vi "{TMPL} MAIN - App.vi"() -> ()   [LabVIEW 2022 SP3, in "TLB` Template.lvlib" / "{TMPL} TLB`.lvclass"]
uses:
  {TMPL} TLB`.lvclass
  Application Components/Trigger API/System Trigger.ctl
  State Machine/State.ctl
  Core Components/Error Handler/TLB` Error Handler.lvclass
  Application Components/Configuration/{TMPL} Station Configuration.lvclass
  {TMPL} TLB`.lvclass/{TMPL} TLB`.ctl
  <vilib>/Utility/error.llb/Error Cluster From Error Code.vi
  <vilib>/ErrorRing/Error Ring.xnode
  Application Components/Trigger API/{TMPL} Trigger API.lvlib
  TLB` Template.lvlib
  Core Components/Actions/Actions.lvlib
  Core Components/Dependencies/TLB`_Dependencies.lvlib
panel:
  out "Banner Text":bool
  in  "Preferences Button":bool=TRUE
  out "Waveform Graph - Light":dbl[](graph)
  in  "Main Tab":T1(tab)
  out "error out":errorcluster
  in  "Connect Instrument":bool
  in  "Disconnect Instrument":bool
  in  "Initiate Analysis":bool
  in  "Stop Analysis":bool
  in  "Load Configuration":bool
  in  "Save Configuration":bool
  in  "Exit":bool
  in  "Active Tab Selector":i32(listbox)
  out "State":string="<Shutdown> "
  out "Status":string
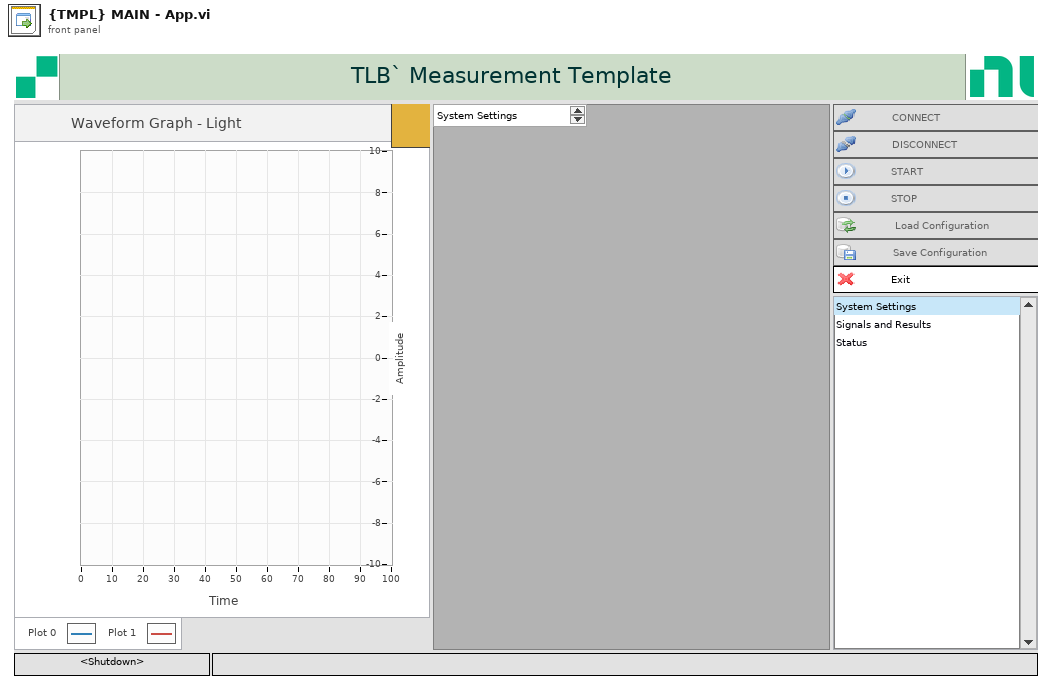
[diagram p1: front panel]
types:
  T1 = enum32{"System Settings", "Signals and Results", "Status"}
  T2 = typedef "TLB` Template.lvlib/{TMPL} TLB`.lvclass/State.ctl" = enum16{"<Startup>", "Idle", "Connected", "Monitoring", "<Shutdown>", "<Error>"}
  T3 = enum16{"Close Display", "Clear References", "Close Error Handler"}
  T4 = enum16{"Clear SR", "Set Display", "Set Shifter", "Initialize Events", "Init Q"}
  T5 = typedef "TLB` Template.lvlib/{TMPL} Trigger API.lvlib/System Trigger.ctl" = enum16{"<None>", "Connect", "Start Acquisition", "Stop Acquisition", "Disconnect", "Load Configuration", "Save Configuration", "<Return to Safe State Actions>", "<Cache User Parameters>", "<Close Application>", "<Error>"}
  T6 = refnum<class "{TMPL} Station Configuration.lvclass">
  T7 = typedef "TLB` Template.lvlib/_UI CORE Event References.ctl" = cluster{"Exit Event":refnum<user-event>, "State Indicator":refnum<user-event>, "Status Indicator":refnum<user-event>}
  T8 = typedef "TLB` Template.lvlib/_UI APP Event References.ctl" = cluster{"Exit Event":refnum<user-event>}
  T9 = enum32{"Invalid", "Standard", "Closed", "Hidden", "Minimized", "Maximized"}
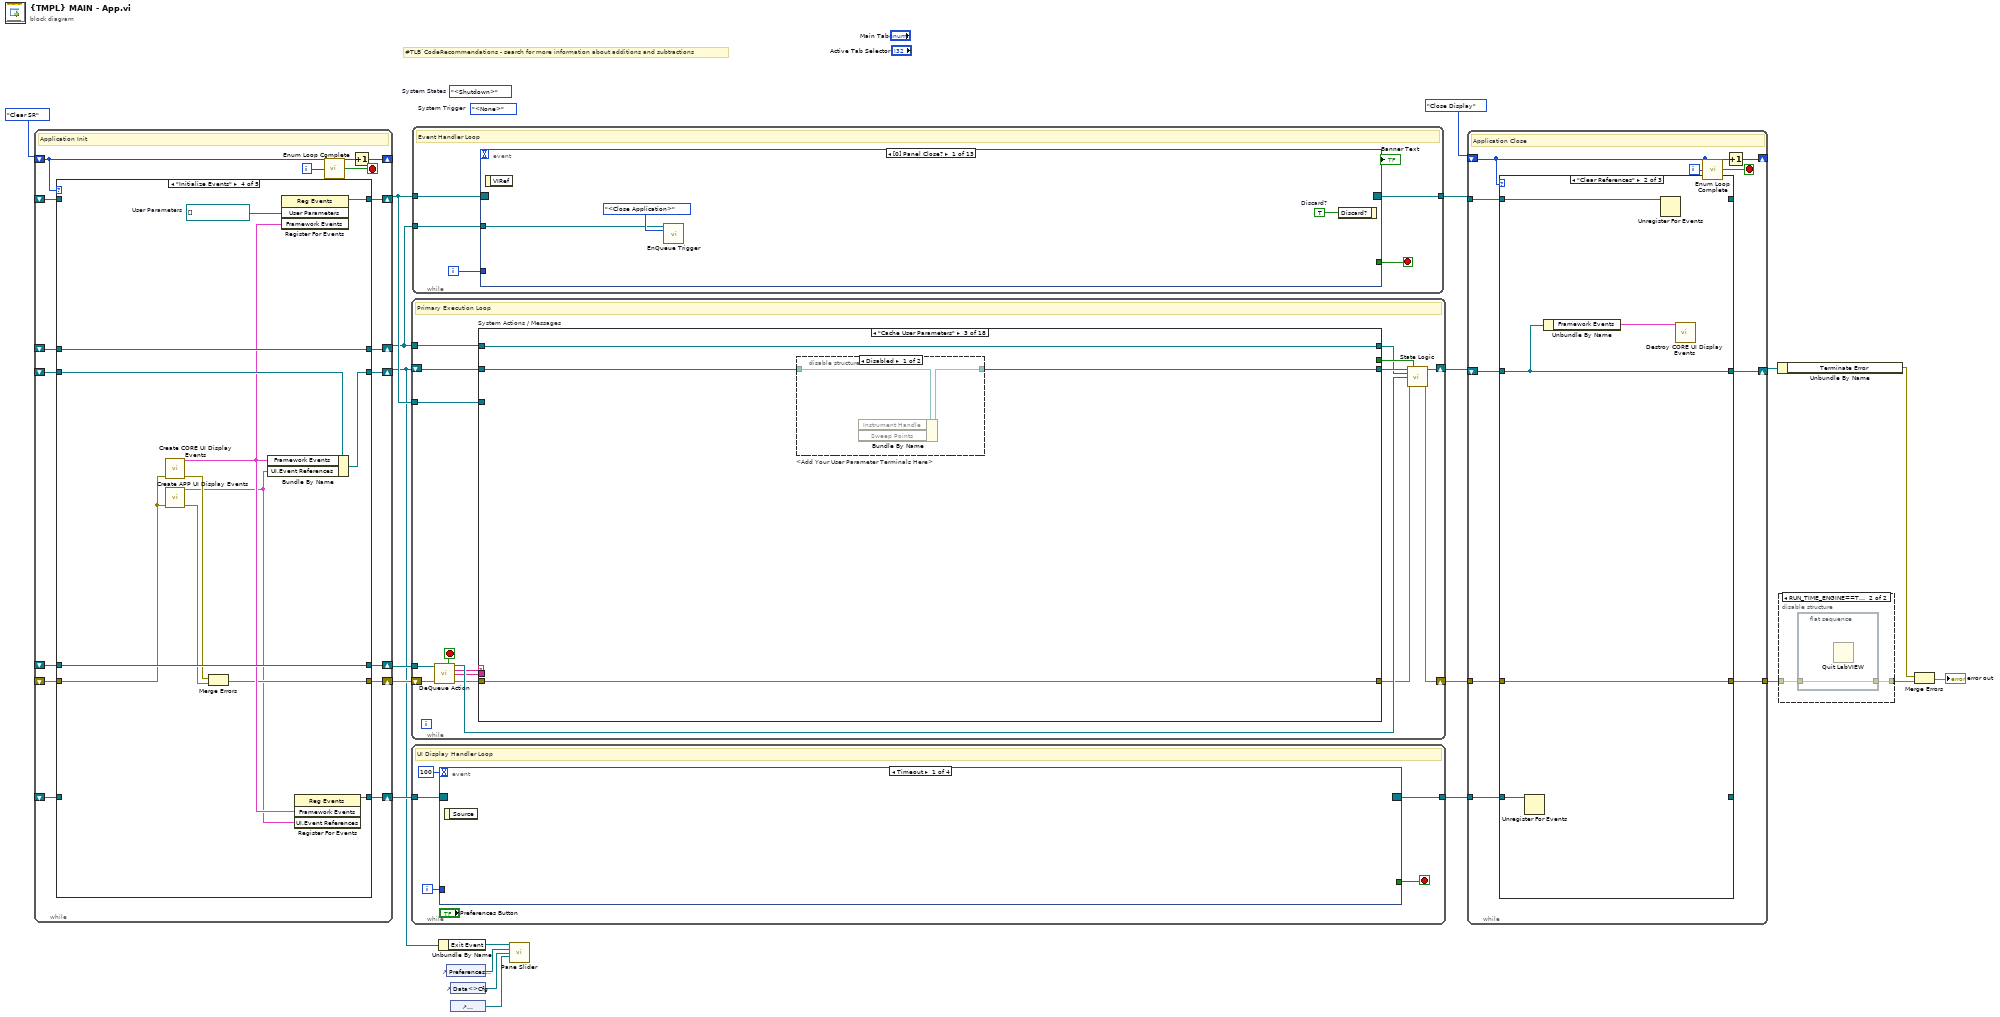
[diagram p0: block diagram]
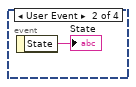
[diagram p2: hidden frame]
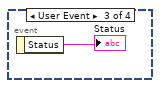
[diagram p3: hidden frame]
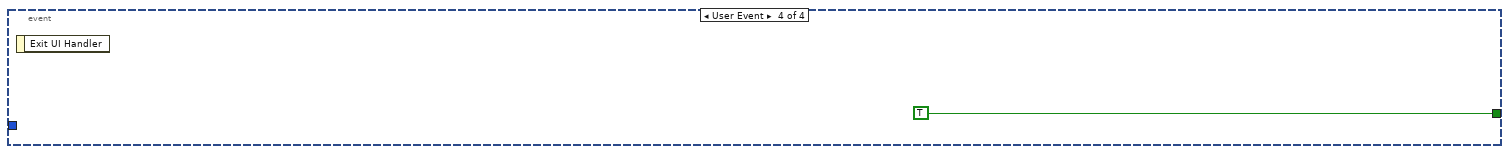
[diagram p4: hidden frame]
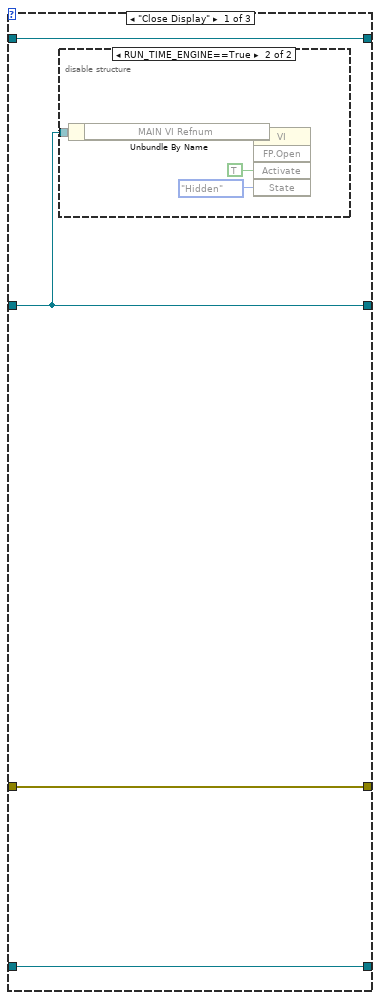
[diagram p6: hidden frame]
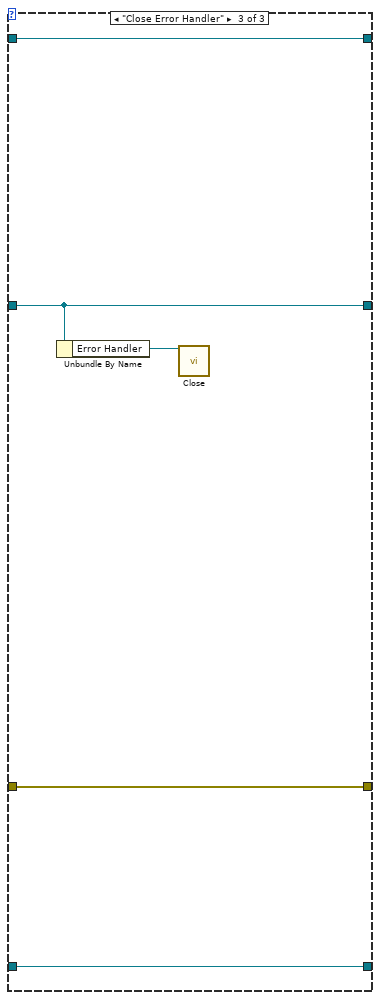
[diagram p8: hidden frame]
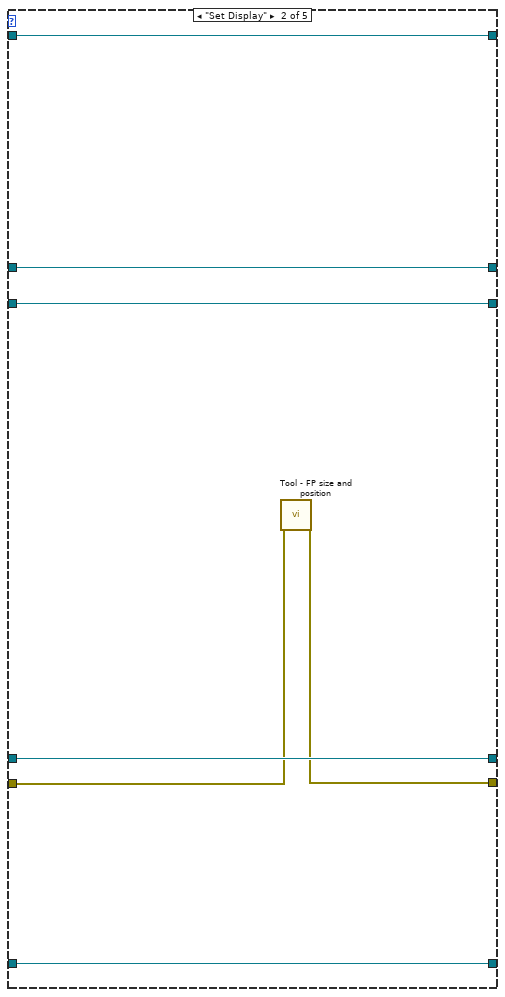
[diagram p10: hidden frame]
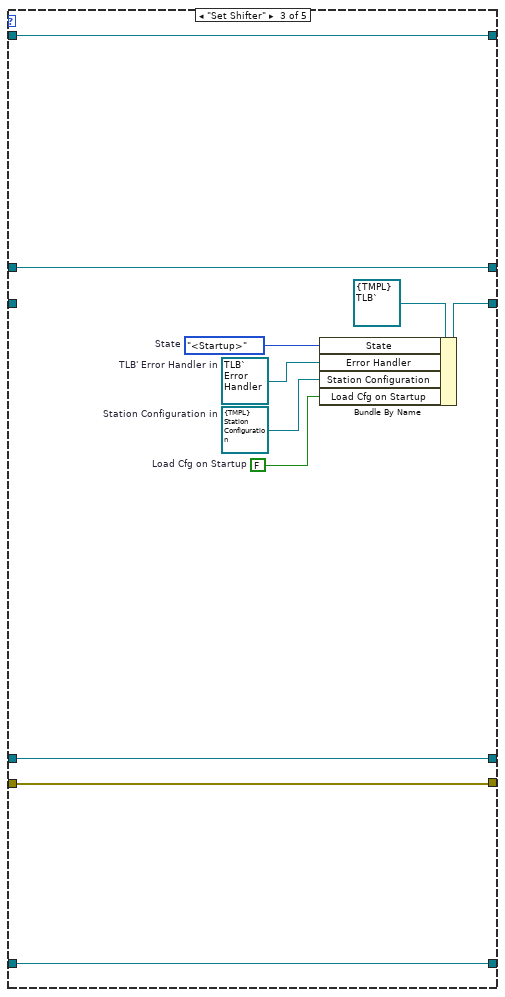
[diagram p11: hidden frame]
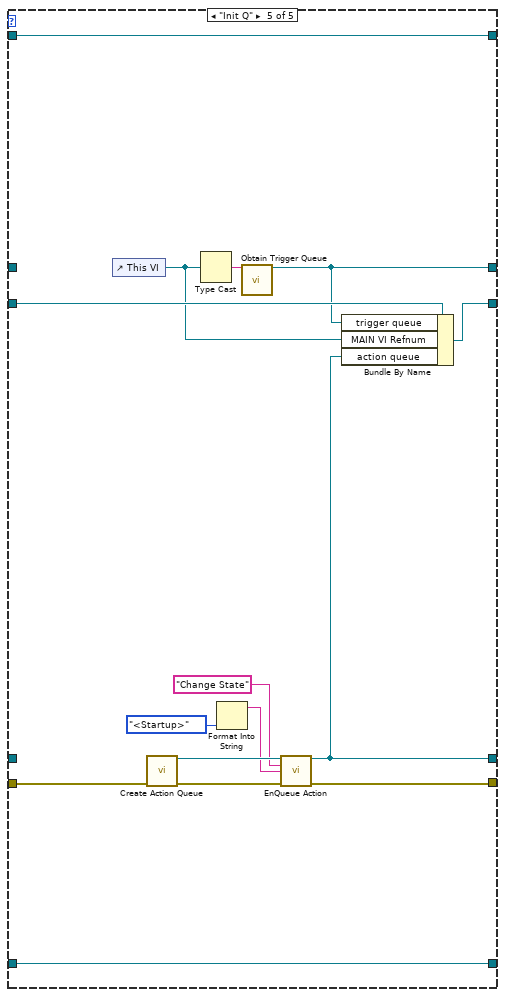
[diagram p12: hidden frame]
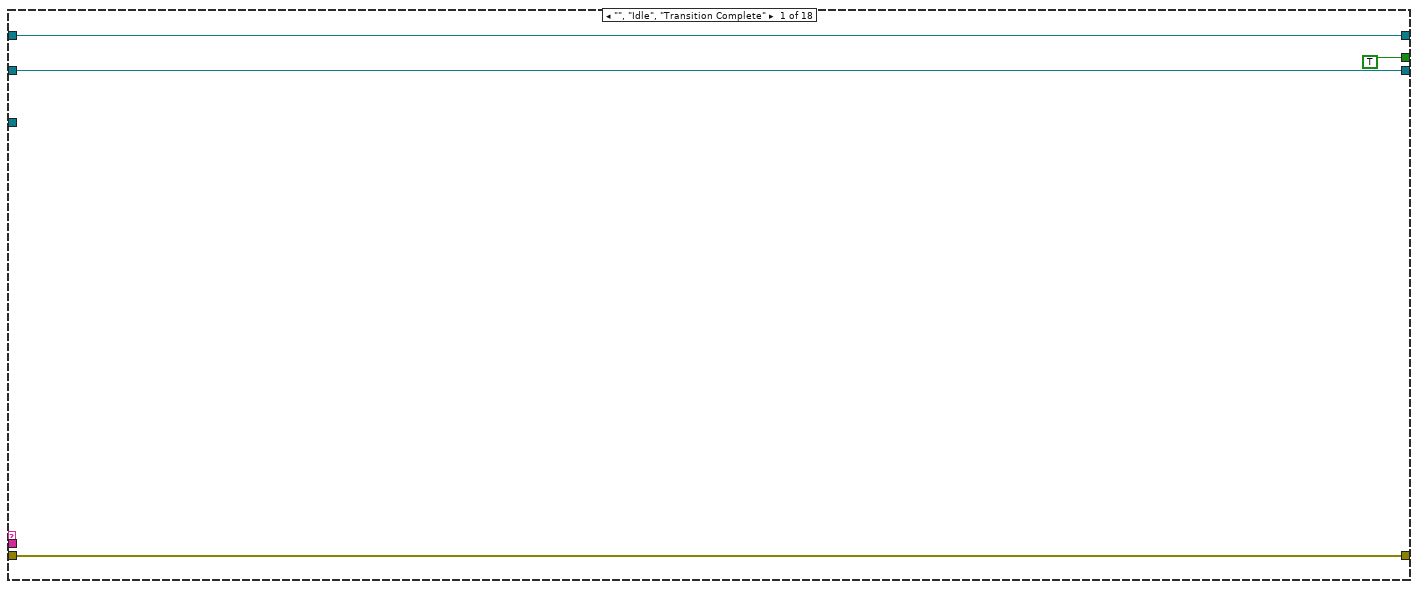
[diagram p13: hidden frame]
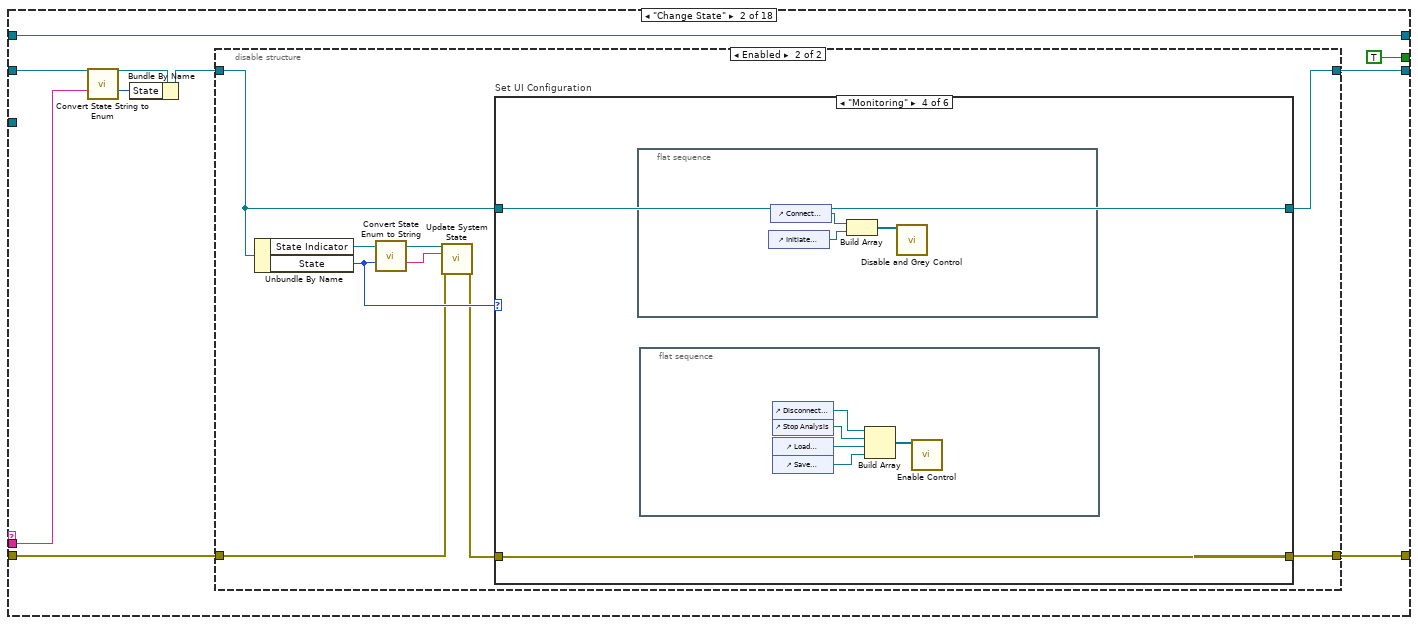
[diagram p14: hidden frame]
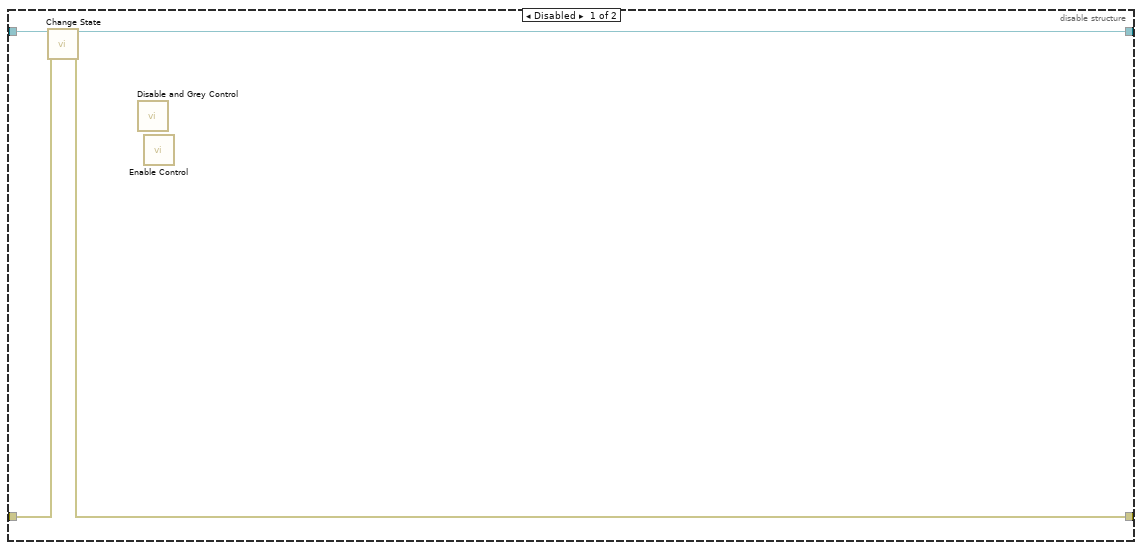
[diagram p15: hidden frame]
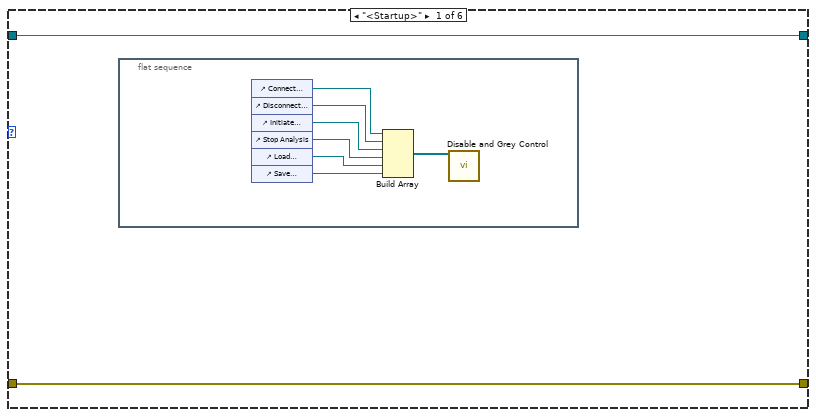
[diagram p16: hidden frame]
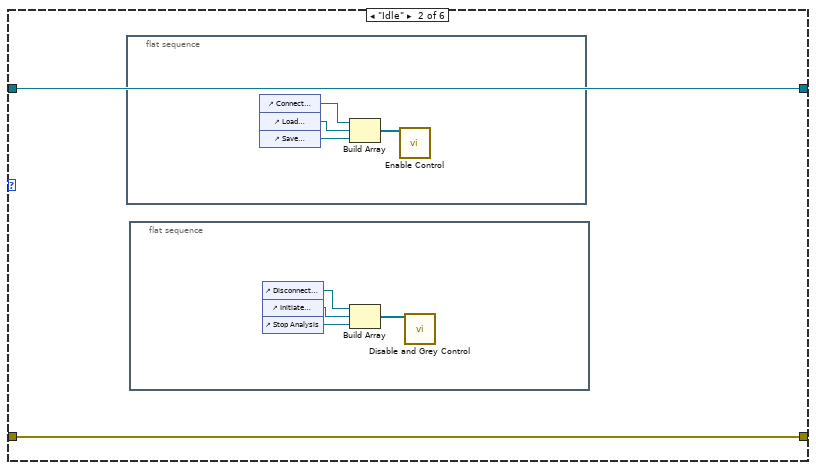
[diagram p17: hidden frame]
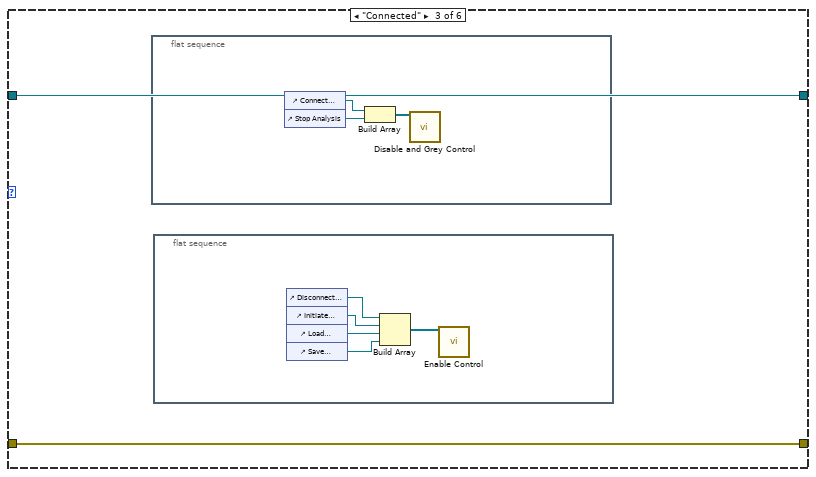
[diagram p18: hidden frame]
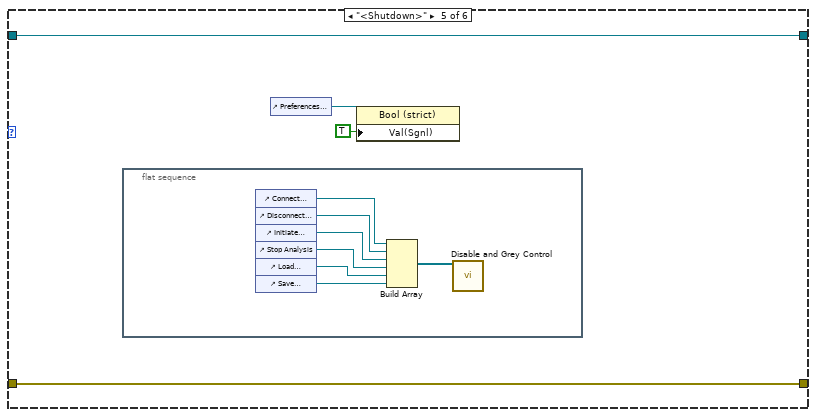
[diagram p19: hidden frame]
diagram:
  (unwired) State."<Shutdown>"  # System States
  (unwired) System_Trigger."<None>"  # System Trigger
  # "#TLB`CodeRecommendations - search for more information about additions and subtractions"
  n1 = while {
    shift-right: [w33] -> _
    shift-left: T4."Clear SR" -> [w22]
    shift-right: [w37] -> w21
    shift-left: _ -> [w32]
    shift-right: [w34] -> w16
    shift-left: _ -> [w31]
    shift-right: [w36] -> w15
    shift-left: _ -> [w30]
    shift-right: [w35] -> w5
    shift-left: _ -> [w29]
    shift-right: [w28] -> w11
    shift-left: _ -> [w27]
    shift-right: [w26] -> w14
    shift-left: _ -> [w25]
    i -> [w23]
    stop <- w24 stop-if-true
    # "Application Init"
    n2 = case shown="\"Initialize Events\"" w22 {
      tunnel: [_ w42 w55 w68 w69] -> w37
      tunnel: [_ w40 w54 w58 w75] -> w34
      tunnel: [_ w44 w50 w66 w81] -> w35
      tunnel: [_ w43 w53 w65 w83] -> w36
      tunnel: w32 -> [_ w42 w55 w68 _]
      tunnel: w31 -> [_ w41 w54 w57 w77]
      tunnel: w30 -> [_ w43 w53 _ w83]
      tunnel: w29 -> [_ w44 _ w67 w82]
      tunnel: [_ w39 w52 w64 w70] -> w28
      tunnel: w27 -> [_ w39 w52 w64 _]
      tunnel: [_ w38 w48 w62 w78] -> w26
      tunnel: w25 -> [_ w38 w48 _ w78]
      frame "Clear SR" {
      }
      frame "Set Display" {
        n3 = call "Tool - FP size and position.vi"("error in (no error)"=w41) -> ("error out"=w40:errorcluster)  [unwired: 17 in, 1 out]
      }
      frame "Set Shifter" {
        w45 = FALSE  # Load Cfg on Startup
        w46 = T6 refnum  # Station Configuration in
        w47 = refnum<class "TLB` Error Handler.lvclass"> refnum  # TLB' Error Handler in
        w51 = State."<Startup>"  # State
        n4 = Bundle By Name(cluster=refnum<class "{TMPL} TLB`.lvclass"> refnum ("TLB` Template.lvlib:TLB' Template.lvclass"), "State"=w51, "Error Handler"=w47, "Station Configuration"=w46, "Load Cfg on Startup"=w45) -> (w50:refnum<class "{TMPL} TLB`.lvclass">)
      }
      frame "Initialize Events" {
        w63 = refnum<vi>[] []  # User Parameters
        n5 = call "Create CORE UI Display Events.vi"("error in"=w57) -> ("Framework Events"=w61:T7, "error out"=w60:errorcluster)  [unwired: 13 in]
        n6 = call "Create APP UI Display Events.vi"("error in"=w57) -> ("UI.Event References"=w56:T8, "error out"=w59:errorcluster)  [unwired: 13 in]
        n7 = Merge Errors(w60, w59) -> (w58:errorcluster)
        n8 = Bundle By Name(cluster=w67, "Framework Events"=w61, "UI.Event References"=w56) -> (w66:refnum<class "{TMPL} TLB`.lvclass">)
        n9 = register-events(w63, w61) -> (reference out=w65:refnum<event-registration>)  [unwired: 2 in, 1 out]
        n10 = register-events(w61, w56) -> (reference out=w62:refnum<event-registration>)  [unwired: 2 in, 1 out]
      }
      frame "Init Q" {
        n11 = control-ref of="This VI"() -> (w80:refnum<vi>)
        n12 = call "Create Action Queue.vi"("error in"=w77) -> ("action queue out"=w74:refnum<queue>, "error out"=w76:errorcluster)  [unwired: 13 in]
        n13 = Type Cast(x=w80) -> (*(type *) &x=w71:string)  [unwired: 1 in]
        n14 = Format Into String(State."<Startup>" ("State")) -> (resulting string=w72:string)  [unwired: 3 in, 1 out]
        n15 = call "Obtain Trigger Queue.vi"("trigger queue name"=w71) -> ("trigger queue out"=w70:refnum<queue>)  [unwired: 13 in, 1 out]
        n16 = call "EnQueue Action.vi"("action queue in"=w74, "action"="Change State" ("Message Name"), "data in"=w72, "error in"=w76) -> ("action queue out"=w69:refnum<queue>, "error out"=w75:errorcluster)  [unwired: 10 in]
        n17 = Bundle By Name(cluster=w82, "trigger queue"=w70, "MAIN VI Refnum"=w80, "action queue"=w69) -> (w81:refnum<class "{TMPL} TLB`.lvclass">)
      }
    }
    n18 = call "Enum Loop Complete.vi"("Current State Enum"=w22, "Itteration"=w23) -> ("Loop Complete?"=w24:bool)  [unwired: 12 in, 1 out]
    n19 = Increment(x=w22) -> (x+1=w33:T4)
  }
  n20 = while {
    shift-right: [w94] -> w13
    shift-left: w16 -> [w89]
    shift-right: [w96] -> w17
    shift-left: w5 -> [w98]
    tunnel: w21 -> [w90]
    tunnel: w15 -> [w97]
    tunnel: w11 -> [w93]
    stop <- w88 stop-if-true
    # "Primary Execution Loop"
    n21 = call "DeQueue Action.vi"("action queue in"=w90, "error in"=w89) -> ("exit?"=w88:bool, "action queue out"=w99:refnum<queue>, "action"=w86:string, "action value"=w84:string, "error out"=w87:errorcluster)  [unwired: 8 in, 1 out]
    n22 = case "System Actions / Messages" shown="\"Cache User Parameters\"" w86 {
      selector: w86 -> [_ _ _ _ _ _ _ _ _ _ _ _ _ _ _ _ _ w274]
      tunnel: [w103 w110 w179 w186 w187 w196 w205 w222 w227 w234 w240 w243 w246 w251 w256 w257 w269 w273] -> w91
      tunnel: w87 -> [w103 w109 w179 w186 w187 w199 w205 w222 w227 w232 w240 w243 w246 w250 w256 w258 w270 _]
      tunnel: w98 -> [w100 w108 w177 w185 w190 w197 w208 w221 w225 w228 w239 w242 w245 w253 w255 w261 w272 w276]
      tunnel: [w100 w104 w180 w185 w189 w202 w211 w221 w225 w229 w239 w242 w245 w253 w255 w260 w271 w276] -> w95
      tunnel: w97 -> [_ _ _ _ _ _ w209 _ _ _ _ _ _ _ _ _ _ _]
      tunnel: [w101 w111 w178 w184 w191 w203 w210 w220 w226 w237 w238 w241 w244 w248 w254 w264 w265 w275] -> w85
      tunnel: w93 -> [w101 w111 w178 w184 w191 w203 w210 w220 w226 w237 w238 w241 w244 w248 w254 w264 w265 w275]
      tunnel: [TRUE TRUE _ _ _ _ _ _ _ _ _ _ _ _ _ _ _ _] -> w92
      tunnel: w84 -> [_ w107 _ _ _ _ _ _ _ _ _ _ _ _ _ _ _ _]
      frame "", "Idle", "Transition Complete" {
      }
      frame "Change State" {
        n23 = call "Convert State String to Enum.vi"("state in"=w107) -> ("state out"=w106:T2)  [unwired: 13 in, 1 out]
        n24 = Bundle By Name(cluster=w108, "State"=w106) -> (w105:refnum<class "{TMPL} TLB`.lvclass">)
        n25 = disable-structure shown="Enabled" {
          disable-tunnel: [w116 w117] -> w110
          disable-tunnel: w109 -> [w115 w118]
          disable-tunnel: w105 -> [w114 w120]
          disable-tunnel: [w113 w119] -> w104
          frame Disabled {
            n26 = call "Change State.vi"("TLB' data in"=w114, "error in"=w115) -> ("TLB' data out"=w113:refnum<class "{TMPL} TLB`.lvclass">, "error out"=w116:errorcluster)  [unwired: 12 in]
            n27 = call "Disable and Grey Control.vi"() -> ()  [unwired: 15 in, 1 out]
            n28 = call "Enable Control.vi"() -> ()  [unwired: 15 in, 1 out]
          }
          frame Enabled {
            n29 = Unbundle By Name(w120) -> ("State Indicator"=w121:refnum<user-event>, "State"=w124:T2)
            n30 = call "Convert State Enum to String.vi"("state in"=w124) -> ("state out"=w122:string)  [unwired: 13 in, 1 out]
            n31 = call "Update System State.vi"("State Indicator"=w121, "system state message"=w122, "error in"=w118) -> ("error out"=w123:errorcluster)  [unwired: 12 in]
            n32 = case "Set UI Configuration" shown="\"Monitoring\"" w124 {
              tunnel: [w125 w135 w145 w155 w167 w175] -> w117
              tunnel: w123 -> [w125 w135 w145 w155 w167 w175]
              tunnel: [w126 w134 w144 w154 w166 w176] -> w119
              tunnel: w120 -> [w126 w134 w144 w154 w166 w176]
              frame "<Startup>" {
                n33 = flat-sequence {
                  frame #0 {
                    n34 = control-ref of="Connect Instrument"() -> (w133:refnum<vi>)
                    n35 = control-ref of="Disconnect Instrument"() -> (w132:refnum<vi>)
                    n36 = control-ref of="Initiate Analysis"() -> (w131:refnum<vi>)
                    n37 = control-ref of="Stop Analysis"() -> (w130:refnum<vi>)
                    n38 = control-ref of="Load Configuration"() -> (w129:refnum<vi>)
                    n39 = control-ref of="Save Configuration"() -> (w128:refnum<vi>)
                    n40 = Build Array(w133, w132, w131, w130, w129, w128) -> (w127:refnum<vi>[])
                    n41 = call "Disable and Grey Control.vi"("Control Ref"=w127) -> ()  [unwired: 14 in, 1 out]
                  }
                }
              }
              frame "Idle" {
                n42 = flat-sequence {
                  frame #0 {
                    n43 = control-ref of="Connect Instrument"() -> (w141:refnum<vi>)
                    n44 = control-ref of="Load Configuration"() -> (w143:refnum<vi>)
                    n45 = control-ref of="Save Configuration"() -> (w142:refnum<vi>)
                    n46 = Build Array(w141, w143, w142) -> (w140:refnum<vi>[])
                    n47 = call "Enable Control.vi"("Control Ref"=w140) -> ()  [unwired: 14 in, 1 out]
                  }
                }
                n48 = flat-sequence {
                  frame #0 {
                    n49 = control-ref of="Disconnect Instrument"() -> (w139:refnum<vi>)
                    n50 = control-ref of="Initiate Analysis"() -> (w138:refnum<vi>)
                    n51 = control-ref of="Stop Analysis"() -> (w137:refnum<vi>)
                    n52 = Build Array(w139, w138, w137) -> (w136:refnum<vi>[])
                    n53 = call "Disable and Grey Control.vi"("Control Ref"=w136) -> ()  [unwired: 14 in, 1 out]
                  }
                }
              }
              frame "Connected" {
                n54 = flat-sequence {
                  frame #0 {
                    n55 = control-ref of="Connect Instrument"() -> (w153:refnum<vi>)
                    n56 = control-ref of="Stop Analysis"() -> (w152:refnum<vi>)
                    n57 = Build Array(w153, w152) -> (w151:refnum<vi>[])
                    n58 = call "Disable and Grey Control.vi"("Control Ref"=w151) -> ()  [unwired: 14 in, 1 out]
                  }
                }
                n59 = flat-sequence {
                  frame #0 {
                    n60 = control-ref of="Disconnect Instrument"() -> (w150:refnum<vi>)
                    n61 = control-ref of="Initiate Analysis"() -> (w149:refnum<vi>)
                    n62 = control-ref of="Load Configuration"() -> (w148:refnum<vi>)
                    n63 = control-ref of="Save Configuration"() -> (w147:refnum<vi>)
                    n64 = Build Array(w150, w149, w148, w147) -> (w146:refnum<vi>[])
                    n65 = call "Enable Control.vi"("Control Ref"=w146) -> ()  [unwired: 14 in, 1 out]
                  }
                }
              }
              frame "Monitoring" {
                n66 = flat-sequence {
                  frame #0 {
                    n67 = control-ref of="Initiate Analysis"() -> (w161:refnum<vi>)
                    n68 = control-ref of="Connect Instrument"() -> (w163:refnum<vi>)
                    n69 = Build Array(w163, w161) -> (w162:refnum<vi>[])
                    n70 = call "Disable and Grey Control.vi"("Control Ref"=w162) -> ()  [unwired: 14 in, 1 out]
                  }
                }
                n71 = flat-sequence {
                  frame #0 {
                    n72 = control-ref of="Disconnect Instrument"() -> (w160:refnum<vi>)
                    n73 = control-ref of="Stop Analysis"() -> (w156:refnum<vi>)
                    n74 = control-ref of="Load Configuration"() -> (w159:refnum<vi>)
                    n75 = control-ref of="Save Configuration"() -> (w158:refnum<vi>)
                    n76 = Build Array(w160, w156, w159, w158) -> (w157:refnum<vi>[])
                    n77 = call "Enable Control.vi"("Control Ref"=w157) -> ()  [unwired: 14 in, 1 out]
                  }
                }
              }
              frame "<Shutdown>" {
                n78 = flat-sequence {
                  frame #0 {
                    n79 = control-ref of="Connect Instrument"() -> (w174:refnum<vi>)
                    n80 = control-ref of="Disconnect Instrument"() -> (w173:refnum<vi>)
                    n81 = control-ref of="Initiate Analysis"() -> (w172:refnum<vi>)
                    n82 = control-ref of="Stop Analysis"() -> (w171:refnum<vi>)
                    n83 = control-ref of="Load Configuration"() -> (w170:refnum<vi>)
                    n84 = control-ref of="Save Configuration"() -> (w169:refnum<vi>)
                    n85 = Build Array(w174, w173, w172, w171, w170, w169) -> (w168:refnum<vi>[])
                    n86 = call "Disable and Grey Control.vi"("Control Ref"=w168) -> ()  [unwired: 14 in, 1 out]
                  }
                }
                n87 = control-ref of="Preferences Button"() -> (w165:refnum<vi>)
                n88 = property class="Bool (strict)"(reference=w165, "Val(Sgnl)"=TRUE ("Value (Signaling)")) -> ()  [unwired: 1 in, 2 out]
              }
              frame "<Error>" {
              }
            }
          }
        }
      }
      frame "Cache User Parameters" {
        n89 = disable-structure "<Add Your User Parameter Terminals Here>" shown="Disabled" {
          disable-tunnel: [w182 w183] -> w180
          disable-tunnel: w177 -> [w181 w183]
          frame Disabled {
            n90 = Bundle By Name(cluster=w181) -> (w182:refnum<class "{TMPL} TLB`.lvclass">)  [unwired: 2 in]
          }
          frame Enabled {
          }
        }
      }
      frame "/*********INITialize********/" {
      }
      frame "INIT::Load Application Base Path" {
        n91 = disable-structure shown="Default" {
          disable-tunnel: [w192 w194] -> w188
          frame condition #0 (active) {
            n92 = Current VI's Path() -> (path=w193:path)
            n93 = Strip Path(path=w193) -> (stripped path=w192:path)  [unwired: 1 out]
          }
          frame condition #1 {
            n94 = call <vilib>:"Application Directory.vi"() -> ("Application Directory"=w194:path)
          }
        }
        n95 = Bundle By Name(cluster=w190, "Application Base Path"=w188) -> (w189:refnum<class "{TMPL} TLB`.lvclass">)
      }
      frame "INIT::Initialize Error Handler" {
        n96 = Unbundle By Name(w197) -> ("Application Base Path"=w204:path)
        n97 = Unbundle By Name(w197) -> ("Error Handler"=w198:refnum<class "TLB` Error Handler.lvclass">)
        n98 = Build Path(base path=w204, name or relative path="System Level Errors\\System Errors.txt") -> (appended path=w200:path)
        n99 = call-dynamic "Open.vi"("error handler in"=w198, "error log path in"=w200, "error in"=w199) -> ("error handler out"=w201:refnum<class "TLB` Error Handler.lvclass">, "error out"=w196:errorcluster)  [unwired: 11 in]
        n100 = Bundle By Name(cluster=w197, "Error Handler"=w201) -> (w202:refnum<class "{TMPL} TLB`.lvclass">)
      }
      frame "INIT::Register User Parameters" {
        n101 = disable-structure shown="Enabled" {
          disable-tunnel: [w212 refnum<vi>[] [] ("User Parameter Controls")] -> w207
          frame Disabled {
            n102 = stacked-sequence "Stacked Sequence Structure :: Allows for a lot of controls" {
              tunnel: [w215] -> w212
              frame #0 {
                n103 = Build Array() -> (w215:void[], w214:dbl, w213:dbl)
              }
            }
          }
          frame Enabled {
          }
        }
        n104 = Build Array (concatenate)(w207) -> (w206:refnum<vi>[])
        n105 = register-events(reference=w209, w206) -> ()  [unwired: 2 in, 2 out]
        n106 = Bundle By Name(cluster=w208, "User Parameter Controls"=w206) -> (w211:refnum<class "{TMPL} TLB`.lvclass">)
      }
      frame "INIT::FP Values" {
        w217 = 0
        # "#TLB`CodeRecommendations - initialize FP values here"
        n107 = property on="Main Tab" class="TabCtl (strict)"() -> ("Pages"=w219:refnum<vi>[])  [unwired: 2 in, 2 out]
        n108 = for {
          tunnel: w219 -> [w224] mode=indexing
          tunnel: [w223] -> w218 mode=indexing
          n109 = property class="Page"(reference=w224) -> ("TabCaption"=w223:string)  [unwired: 1 in, 2 out]
        }
        n110 = property on="Active Tab Selector" class="LstBox (strict)"("Item Names"=w218) -> ()  [unwired: 2 in, 2 out]
        n111 = local write "Active Tab Selector"(w217) -> ()
        n112 = local write "Main Tab"(w217) -> ()
      }
      frame "INIT::Initialize System Parameters" {
      }
      frame "CFG::Load Station Configuration" {
        n113 = Unbundle By Name(w228) -> ("Station Configuration"=w231:T6)
        n114 = Unbundle By Name(w228) -> ("Application Base Path"=w236:path)
        n115 = Build Path(base path=w236, name or relative path="System Configuration\\Station Configuration.ini") -> (appended path=w233:path)
        n116 = call-dynamic "Load Configuration.vi"("INI Station Configuration in"=w231, "INI file path in"=w233, "error in"=w232) -> ("INI Station Configuration out"=w230:T6, "error out"=w234:errorcluster)  [unwired: 11 in]
        n117 = Bundle By Name(cluster=w228, "Station Configuration"=w230) -> (w229:refnum<class "{TMPL} TLB`.lvclass">)
      }
      frame "/*********PRImary EXEcution********/" {
      }
      frame "APP::Update Display" {
      }
      frame "/*********SHUTDOWN********/" {
      }
      frame "Exit" {
        w249 = refnum<class> refnum  # event data
        # "Don't wire 'Error In'\nMust Execute Regardless"
        n118 = Unbundle By Name(w253) -> ("Exit Event"=w247:refnum<user-event>)
        n119 = Generate User Event(user event=w247, event data cluster=w249) -> (error out=w252:errorcluster)  [unwired: 2 in, 1 out]
        n120 = Merge Errors(w250, w252) -> (w251:errorcluster)
      }
      frame "/*********ERRor Handler********/" {
      }
      frame "ERR::Log" {
        n121 = Unbundle By Name(w261) -> ("Error Handler"=w263:refnum<class "TLB` Error Handler.lvclass">)
        n122 = call-dynamic "Log.vi"("error handler in"=w263) -> ("error handler out"=w262:refnum<class "TLB` Error Handler.lvclass">, "error out"=w259:errorcluster)  [unwired: 13 in]
        n123 = Bundle By Name(cluster=w261, "Error Handler"=w262) -> (w260:refnum<class "{TMPL} TLB`.lvclass">)
        n124 = Merge Errors(w258, w259) -> (w257:errorcluster)
      }
      frame "ERR::Dialog" {
        n125 = Unbundle By Name(w272) -> ("Error Handler"=w268:refnum<class "TLB` Error Handler.lvclass">)
        n126 = call-dynamic "Dialog.vi"("error handler in"=w268, "trigger queue in"=w265) -> ("error handler out"=w267:refnum<class "TLB` Error Handler.lvclass">, "error out"=w266:errorcluster)  [unwired: 12 in]
        n127 = Merge Errors(w270, w266) -> (w269:errorcluster)
        n128 = Bundle By Name(cluster=w272, "Error Handler"=w267) -> (w271:refnum<class "{TMPL} TLB`.lvclass">)
      }
      frame Default {
        n129 = xnode "Error Ring"("parameter 0"=w274) -> ("error out"=w273:errorcluster)
      }
    }
    n130 = call "State Logic.vi"("TLB' data in"=w95, "process state logic enable"=w92, "trigger queue in"=w85, "action queue in"=w99, "error in"=w91) -> ("TLB' data out"=w96:refnum<class "{TMPL} TLB`.lvclass">, "error out"=w94:errorcluster)  [unwired: 9 in]
  }
  n131 = while {
    tunnel: w14 -> [w288]
    tunnel: [w284] -> w12
    i -> [w287]
    stop <- w286 stop-if-true
    # "UI Display Handler Loop"
    n132 = event shown="[0] Timeout" {
      selector: w288 -> [_ _ _ _]
      dyn-events: [_ _ _ _] -> w284
      timeout: 100 -> [_ _ _ _]
      tunnel: w287 -> [_ _ _ _]
      tunnel: [_ _ _ TRUE] -> w286
      event Timeout {
        n133 = event-data() -> ()  [unwired: 2 out]
      }
      event User Event {
        n134 = event-data() -> ("State"=→"State":string)  [unwired: 1 out]
      }
      event User Event {
        n135 = event-data() -> ("Status"=→"Status":string)  [unwired: 1 out]
      }
      event User Event {
        n136 = event-data() -> ()  [unwired: 2 out]
      }
    }
  }
  n137 = while {
    tunnel: w15 -> [w295]
    tunnel: [w294] -> w18
    tunnel: w11 -> [w292]
    i -> [w293]
    stop <- w296 stop-if-true
    # "Event Handler Loop"
    n138 = event shown="[0] Panel Close?" {
      selector: w295 -> [_ _ _ _ _ _ _ _ _ _ _ _ _]
      dyn-events: [_ _ _ _ _ _ _ _ _ _ _ _ _] -> w294
      timeout: _ -> [_ _ _ _ _ _ _ _ _ _ _ _ _]
      tunnel: [_ _ TRUE ("NewVal") _ _ _ _ _ _ _ _ _ _] -> w296
      tunnel: w293 -> [_ _ _ _ _ _ _ _ _ _ _ _ _]
      tunnel: w292 -> [w297 _ w309 w313 w316 w318 w320 w322 w324 w326 w327 _ _]
      event Panel Close? {
        w299 = TRUE  # Discard?
        n139 = event-data() -> ()  [unwired: 2 out]
        n140 = call "EnQueue Trigger.vi"("trigger queue in"=w297, "system trigger"=System_Trigger."<Close Application>" ("System Trigger")) -> ()  [unwired: 12 in, 2 out]
        n141 = event-data("Discard?"=w299) -> ()  [unwired: 1 in, 1 out]
      }
      event Mouse Down {
        n142 = event-data() -> ("Button"=w300:u16, "Mods.Double Click"=w301:bool)  [unwired: 1 out]
        n143 = Equal?(x=u16 2, y=w300) -> (x = y?=w303:bool)
        n144 = Compound Arithmetic op=AND(w303, w301) -> (w302:bool)
        n145 = case "Toggle Menu Visibility :: double RIGHT click on logo" shown="True" w302 {
          frame False {
          }
          frame True {
            n146 = property class="VI"() -> (reference out=w307:refnum<vi>, "TB.Visible"=w306:bool)  [unwired: 2 in, 1 out]
            n147 = Not(x=w306) -> (.not. x?=w305:bool)
            n148 = property class="VI"(reference=w307, "TB.Visible"=w305, "Front Panel.ShowMenuBar"=w305) -> ()  [unwired: 1 in, 2 out]
          }
        }
      }
      event User Event {
        n149 = event-data() -> ()  [unwired: 2 out]
        n150 = call "EnQueue Trigger.vi"("trigger queue in"=w309, "system trigger"=System_Trigger."<Close Application>" ("System Trigger")) -> ()  [unwired: 12 in, 2 out]
      }
      event Value Change {
        n151 = event-data() -> ()  [unwired: 2 out]
        n152 = call "EnQueue Trigger.vi"("trigger queue in"=w313, "system trigger"=System_Trigger."<Cache User Parameters>" ("System Trigger")) -> ("trigger queue out"=w312:refnum<queue>)  [unwired: 12 in, 1 out]
        n153 = event "use this event case to register a SPEICIFIC 'User Parameter' for a SPECIFIC action" shown="[0] Timeout" {
          selector: _ -> [_]
          dyn-events: _ -> [_]
          timeout: 0 -> [_]
          tunnel: w312 -> [_]
          event Timeout {
            n154 = event-data() -> ()  [unwired: 1 in, 1 out]
          }
        }
      }
      event "Connect Instrument": Value Change {
        n155 = event-data() -> ()  [unwired: 2 out]
        n156 = call "EnQueue Trigger.vi"("trigger queue in"=w316, "system trigger"=System_Trigger."Connect" ("System Trigger")) -> ()  [unwired: 12 in, 2 out]
      }
      event "Disconnect Instrument": Value Change {
        n157 = event-data() -> ()  [unwired: 2 out]
        n158 = call "EnQueue Trigger.vi"("trigger queue in"=w318, "system trigger"=System_Trigger."Disconnect" ("System Trigger")) -> ()  [unwired: 12 in, 2 out]
      }
      event "Initiate Analysis": Value Change {
        n159 = event-data() -> ()  [unwired: 2 out]
        n160 = call "EnQueue Trigger.vi"("trigger queue in"=w320, "system trigger"=System_Trigger."Start Acquisition" ("System Trigger")) -> ()  [unwired: 12 in, 2 out]
      }
      event "Stop Analysis": Value Change {
        n161 = event-data() -> ()  [unwired: 2 out]
        n162 = call "EnQueue Trigger.vi"("trigger queue in"=w322, "system trigger"=System_Trigger."Stop Acquisition" ("System Trigger")) -> ()  [unwired: 12 in, 2 out]
      }
      event "Save Configuration": Value Change {
        n163 = event-data() -> ()  [unwired: 2 out]
        n164 = call "EnQueue Trigger.vi"("trigger queue in"=w324, "system trigger"=System_Trigger."Save Configuration" ("System Trigger")) -> ()  [unwired: 12 in, 2 out]
      }
      event "Load Configuration": Value Change {
        n165 = event-data() -> ()  [unwired: 2 out]
        n166 = call "EnQueue Trigger.vi"("trigger queue in"=w326, "system trigger"=System_Trigger."Load Configuration" ("System Trigger")) -> ()  [unwired: 12 in, 2 out]
      }
      event "Exit": Value Change {
        n167 = event-data() -> ()  [unwired: 2 out]
        n168 = call "EnQueue Trigger.vi"("trigger queue in"=w327, "system trigger"=System_Trigger."<Close Application>" ("System Trigger")) -> ()  [unwired: 12 in, 2 out]
      }
      event "Active Tab Selector": Value Change {
        n169 = event-data() -> ("NewVal"=w329:i32)  [unwired: 1 out]
        n170 = local write "Main Tab"(w329) -> ()
      }
      event "Main Tab": Value Change {
        n171 = event-data() -> ("NewVal"=w330:T1)  [unwired: 1 out]
        n172 = local write "Active Tab Selector"(w330) -> ()
      }
    }
  }
  n173 = Unbundle By Name(w5) -> ("Exit Event"=w4:refnum<user-event>)
  n174 = control-ref of="Preferences Button"() -> (w3:refnum<vi>)
  n175 = control-ref of="Data<>Cfg"() -> (w2:refnum<vi>)
  n176 = control-ref of="Cfg<>Control"() -> (w1:refnum<vi>)
  n177 = call "Pane Slider.vi"("User Event in"=w4, "Invoke Button"=w3, "Moving Splitter"=w2, "Fixed Splitter"=w1) -> ()  [unwired: 12 in]
  n178 = while {
    shift-right: [w340] -> _
    shift-left: T3."Close Display" -> [w333]
    tunnel: w18 -> [w338]
    tunnel: w13 -> [w339]
    tunnel: [w336] -> w20
    shift-right: [w335] -> w9
    shift-left: w17 -> [w337]
    tunnel: w12 -> [w334]
    i -> [w331]
    stop <- w332 stop-if-true
    # "Application Close"
    n179 = case shown="\"Clear References\"" w333 {
      tunnel: [w343 w353 w358] -> w336
      tunnel: [w342 w352 w355] -> w335
      tunnel: [w344 _ w357] -> _
      tunnel: w339 -> [w343 w353 w358]
      tunnel: w338 -> [w344 w351 w357]
      tunnel: w337 -> [w342 w352 w355]
      tunnel: w334 -> [w341 w349 w356]
      tunnel: [w341 _ w356] -> _
      frame "Close Display" {
        n180 = disable-structure shown="RUN_TIME_ENGINE==True" {
          disable-tunnel: w342 -> [_ w346]
          frame condition #0 (active) {
          }
          frame condition #1 {
            n181 = Unbundle By Name(w346) -> ("MAIN VI Refnum"=w345:refnum<vi>)
            n182 = invoke class="VI" method="FP.Open"(reference=w345, "Activate"=TRUE ("Activate?"), "State"=T9."Hidden") -> ()  [unwired: 2 in, 5 out]
          }
        }
      }
      frame "Clear References" {
        n183 = Unregister For Events(event registration refnum=w349) -> ()  [unwired: 1 in, 1 out]
        n184 = Unbundle By Name(w352) -> ("Framework Events"=w350:T7)
        n185 = Unregister For Events(event registration refnum=w351) -> ()  [unwired: 1 in, 1 out]
        n186 = call "Destroy CORE UI Display Events.vi"("UI display events in"=w350) -> ()  [unwired: 14 in, 1 out]
      }
      frame "Close Error Handler" {
        n187 = Unbundle By Name(w355) -> ("Error Handler"=w354:refnum<class "TLB` Error Handler.lvclass">)
        n188 = call-dynamic "Close.vi"("error handler in"=w354) -> ()  [unwired: 14 in, 1 out]
      }
    }
    n189 = call "Enum Loop Complete.vi"("Current State Enum"=w333, "Itteration"=w331) -> ("Loop Complete?"=w332:bool)  [unwired: 12 in, 1 out]
    n190 = Increment(x=w333) -> (x+1=w340:T3)
  }
  n191 = Unbundle By Name(w9) -> ("Terminate Error"=w8:errorcluster)
  n192 = disable-structure shown="RUN_TIME_ENGINE==True" {
    disable-tunnel: [w359 w360] -> w7
    disable-tunnel: w20 -> [w359 w361]
    frame condition #0 (active) {
    }
    frame condition #1 {
      n193 = flat-sequence {
        tunnel: [w362] -> w360
        tunnel: w361 -> [w362]
        frame #0 {
          n194 = Quit LabVIEW() -> ()  [unwired: 1 in]
        }
      }
    }
  }
  n195 = Merge Errors(w8, w7) -> (→"error out":errorcluster)
